vi "Generate Data Configuration.vi"(8 "error in (no error)":errorcluster, 10 "Cluster or Array String":string, 11 "Data":variant) -> (0 "error out":errorcluster, 3 "Data Configuration":T1)   [LabVIEW 2021, in "CIF_Iceoryx_BB.lvclass"]
uses:
  CIF_Iceoryx_BB.lvclass
  CIF_Iceoryx_BB.lvclass/CIF_Iceoryx_BB.ctl
  Typedef/Data Configuration.ctl
  <vilib>/CIF Foundation/CIF Iceoryx/Iceoryx.lvlib
  <vilib>/CIF Foundation/CIF Utilities/DataTypes/DataTypes_CIF_U.lvlib
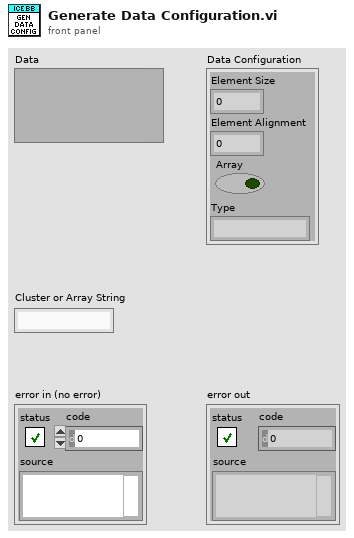
[diagram p1: front panel]
types:
  T1 = typedef "CIF_Iceoryx_BB.lvclass/Data Configuration.ctl" = cluster{"Element Size":u32, "Element Alignment":u32, "Array":bool, "Type":string}
  T2 = typedef "DataTypes_CIF_U.lvlib/Cluster Info.ctl" = cluster{"Name":string[], "Indices":i32[], "Type":T3, "Flat Data Size":u32, "Flat Data Offset":u32, "Memory Size":u32, "Memory Padding":u32, "Memory Offset":u32, "Type Descriptor":i16[]}
  T3 = typedef "NI_Data Type.lvlib/Data Type.ctl" = enum8{"Invalid Type", "Void", "I8", "I16", "I32", "I64", "U8", "U16", "U32", "U64", "Single Float", "Double Float", "Extended Float", "Single Complex", "Double Complex", "Extended Complex", "Enum U8", "Enum U16", "Enum U32", "Enum U64", "Single Float With Unit", "Double Float With Unit", "Extended Float With Unit", "Single Complex with Unit", "Double Complex with Unit", "Extended Complex with Unit", "Boolean", "String", "Path", "Picture", "Tag", "Array", "Cluster", "Variant", "LV Variant", "Waveform", "Timestamp", "Digital Waveform", "Digital Data", "ExpressData", "Refnum", "External Data", "VI", "Poly VI", "LabVIEW Class Instance", "Fixed Point", "Set Collection", "Map Collection"}
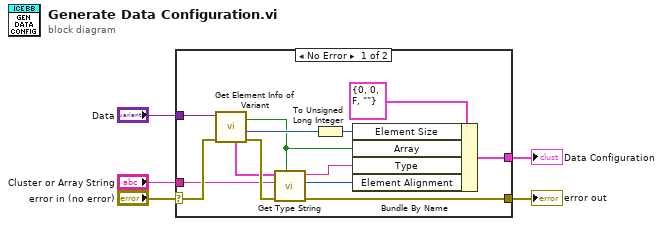
[diagram p0: block diagram]
diagram:
  n1 = case shown="No Error" "error in (no error)" {
    selector: "error in (no error)" -> [w11 w19]
    tunnel: [w12 w19] -> w4
    tunnel: "Data" -> [w10 _]
    tunnel: [w9 _] -> w1
    tunnel: "Cluster or Array String" -> [w7 _]
    frame No Error {
      n2 = call <vilib>:"Get Element Info of Variant.vi"("error in (no error)"=w11, "Data Type"=w10) -> ("error out"=w18:errorcluster, "Array Element Size"=w17:i32, "Cluster Info"=w16:T2[], "Array"=w15:bool)  [unwired: 4 in, 2 out]
      n3 = call <vilib>:"Get Type String.vi"("Array"=w15, "error in (no error)"=w18, "Cluster or Array String"=w7, "Cluster Info"=w16) -> ("error out"=w12:errorcluster, "elem_align"=w13:u32, "Type String"=w8:string)  [unwired: 5 in]
      n4 = To Unsigned Long Integer(number=w17) -> (unsigned 32bit integer=w14:u32)
      n5 = Bundle By Name(cluster=T1 {"Element Size"=0, "Element Alignment"=0, "Array"=FALSE, "Type"=""} ("Data Configuration"), "Element Size"=w14, "Array"=w15, "Type"=w8, "Element Alignment"=w13) -> (w9:T1)
    }
    frame Error {
    }
  }
  "error out" <- w4
  "Data Configuration" <- w1
